vi "Exp - Get VC Handle.vi"(6 "error in":bool, 9 "InstanceRef":T2) -> (0 "error out":bool, 1 "writer ID":u32, 3 "dup InstanceRef":T2, 4 "VC Handle":T1=-1)   [LabVIEW 2021]
doc: "This VI returns the <b>VC Handle</b> and the <b>writer ID</b> associated with the running CalcExpress instance. Refer to the VI help for more details.\n\n::: CalcExpress Toolkit :::\nCopyright (c) 2000-2026 Konstantin Shifershteyn. All rights reserved."
uses:
  cetypes.llb/CalcExpress Instance RefNum.ctl
  cetypes.llb/VarMan Variable Context Handle.ctl
  cersrc/celveng32.dll
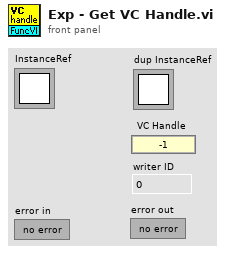
[diagram p1: front panel]
types:
  T1 = typedef "VarMan Variable Context Handle.ctl" = i32
  T2 = typedef "CalcExpress Instance RefNum.ctl" = refnum<k1>
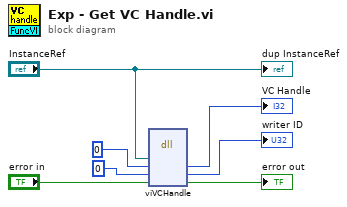
[diagram p0: block diagram]
diagram:
  n1 = dll-call lib="C:/LV Projects/CalcExpress 40 LV2021/vi.lib/addons/CalcExpress/cersrc/celveng*.dll" fn="viVCHandle"("iRef"="InstanceRef", "vch"=0 ("VC Handle"), "writerID"=u32 0, "erf"="error in") -> ("vch"=→"VC Handle":i32, "writerID"=→"writer ID":u32, "erf"=→"error out":bool)  [unwired: 5 in, 2 out]
  "dup InstanceRef" <- "InstanceRef"
